vi "test_PinAndPinGroupContainingSamePin_ReserveSessions_ChannelMappingsDoesNotContainDuplicatePins.vi"() -> (6 "pass":bool, 8 "result":string, 15 "error out":errorcluster)   [LabVIEW 2021, in "MeasurementServerTests.lvlib" / "Session Reservation Tests.lvlib"]
uses:
  Session Reservation Tests.lvlib
  gRPC/Generated APIs/ni/measurementlink/sessionmanagement/v1/RPC Messages/ni_measurementlink_PinMapContext.ctl
  gRPC/Generated APIs/ni/measurementlink/sessionmanagement/v1/RPC Messages/ni_measurementlink_sessionmanagement_v1_ChannelMapping.ctl
  Runtime/Clients/Session Management V1/Session Reservation/Session Reservation.lvclass/Session Reservation.ctl
  3347d1b6-dca7-4e1a-9ca0-c9ec2f5aba95.vi
  ab61e54b-70f9-4719-86d2-c3025959eeb5.vi
  Runtime/Clients/Session Management V1/Session Reservation/Merge Invalid DVR Error.vi
  Runtime/Clients/Session Management V1/Session Reservation/Is DVR Valid.vi
  Runtime/Measurements/Helpers/Error Strings Global Internal.vi
  <vilib>/Utility/error.llb/Error Cluster From Error Code.vi
  <vilib>/JDP Science/JSONtext/Variant to JSON Text.vi
  <vilib>/JDP Science/JSONtext/LVClass Serializer/JSONtext LVClass Serializer.lvclass
  gRPC/Generated APIs/ni/measurementlink/sessionmanagement/v1/ni.measurementlink.sessionmanagement.v1.api.lvlib
  MeasurementServerTests.lvlib
  Runtime/Clients/Session Management V1/Session Reservation/Session Reservation.lvclass
panel:
  # "Test assumes discovery service, pin map service, and session management service have already been started."
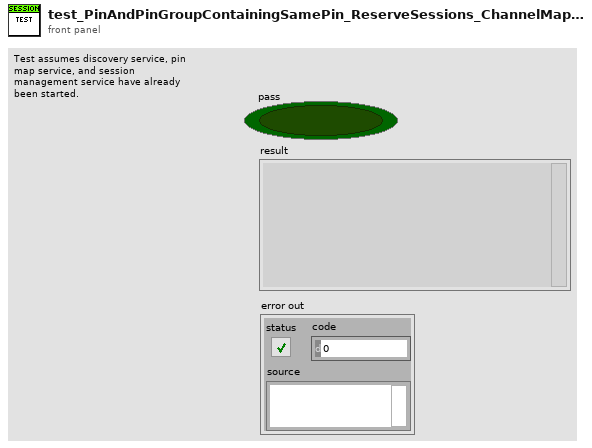
[diagram p1: front panel]
types:
  T1 = typedef "ni.measurementlink.sessionmanagement.v1.api.lvlib/ni_measurementlink_sessionmanagement_v1_ChannelMapping.ctl" = cluster{"pin_or_relay_name":string, "site":i32, "channel":string, "multiplexer_resource_name":string, "multiplexer_route":string}
  T2 = typedef "ni.measurementlink.sessionmanagement.v1.api.lvlib/ni_measurementlink_PinMapContext.ctl" = cluster{"pin_map_id":string, "sites":i32[]}
  T3 = typedef "ni.measurementlink.sessionmanagement.v1.api.lvlib/ni_measurementlink_sessionmanagement_v1_SessionInformation.ctl" = cluster{"session":T4, "resource_name":string, "channel_list":string, "instrument_type_id":string, "session_exists":bool, "session_reserved":bool, "channel_mappings":T1[], "annotations":T5[]}
  T4 = typedef "ni.measurementlink.sessionmanagement.v1.api.lvlib/nidevice_grpc_Session.ctl" = cluster{"name":string}
  T5 = typedef "ni.measurementlink.sessionmanagement.v1.api.lvlib/ni_measurementlink_sessionmanagement_v1_SessionInformation_AnnotationsEntry.ctl" = cluster{"key":string, "value":string}
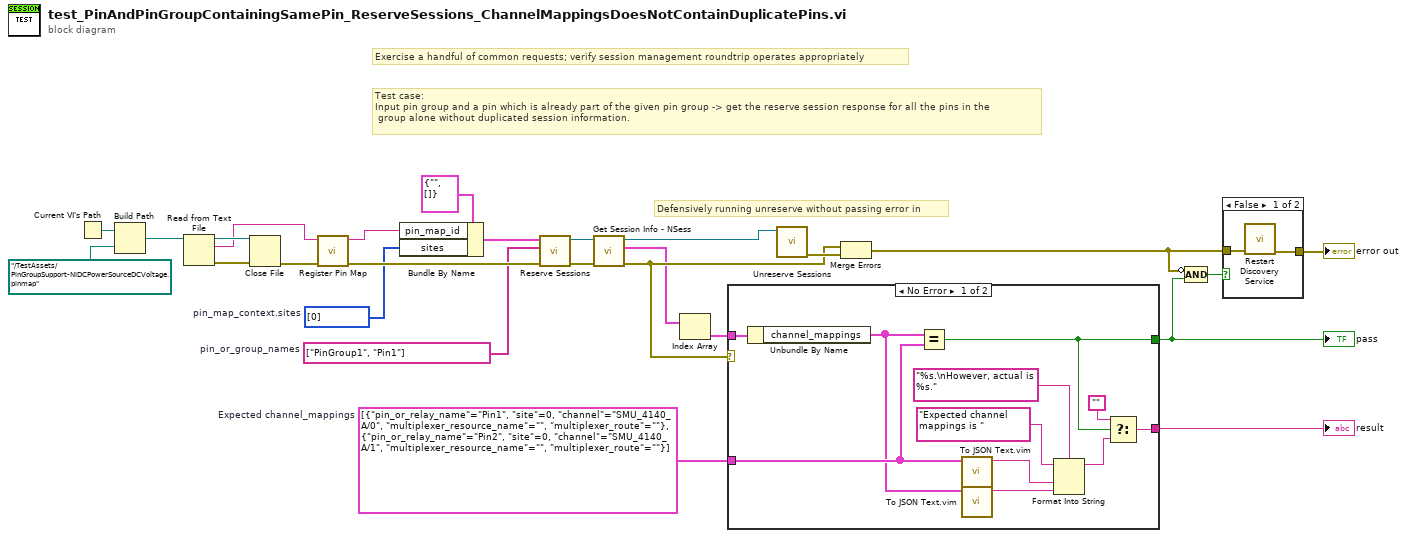
[diagram p0: block diagram]
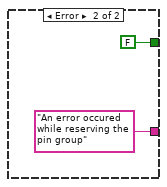
[diagram p3: hidden frame]
diagram:
  w5 = T1[] [{"pin_or_relay_name"="Pin1", "site"=0, "channel"="SMU_4140_A/0", "multiplexer_resource_name"="", "multiplexer_route"=""}, {"pin_or_relay_name"="Pin2", "site"=0, "channel"="SMU_4140_A/1", "multiplexer_resource_name"="", "multiplexer_route"=""}]  # Expected channel_mappings
  w10 = i32[] [0]  # pin_map_context.sites
  w9 = string[] ["PinGroup1", "Pin1"]  # pin_or_group_names
  # "Defensively running unreserve without passing error in"
  # "Test case:\nInput pin group and a pin which is already part of the given pin group -> get the reserve session response for all the pins in the\n\tgroup alone without duplicated session information."
  # "Exercise a handful of common requests; verify session management roundtrip operates appropriately"
  n1 = Current VI's Path() -> (path=w26:path)
  n2 = Build Path(base path=w26, name or relative path=path "../TestAssets/PinGroupSupport-NIDCPowerSourceDCVoltage.pinmap") -> (appended path=w24:path)
  n3 = Read from Text File(file (use dialog)=w24) -> (refnum out=w22:refnum<file>, text=w20:string, error out=w23:errorcluster)  [unwired: 3 in, 1 out]
  n4 = Close File(refnum=w22, error in=w23) -> (error out=w8:errorcluster)  [unwired: 1 out]
  n5 = call "Register Pin Map.vi"("error in"=w8, "pin map xml"=w20) -> ("error out"=w12:errorcluster, "pin map id"=w11:string)  [unwired: 8 in]
  n6 = Bundle By Name(cluster=T2 {"pin_map_id"="", "sites"=[]} ("pin map context"), "pin_map_id"=w11, "sites"=w10) -> (w19:T2)
  n7 = call "Reserve Sessions.vi"("error in"=w12, "pin or relay names"=w9, "pin map context"=w19) -> ("error out"=w18:errorcluster, "session reservation out"=w17:refnum<class "Session Reservation.lvclass">)  [unwired: 7 in]
  n8 = call "Get Session Info - NSess .vi"("error in"=w18, "session reservation in"=w17) -> ("error out"=w13:errorcluster, "sessions info"=w7:T3[], "session reservation out"=w6:refnum<class "Session Reservation.lvclass">)  [unwired: 7 in]
  n9 = Index Array(array=w7) -> (element=w1:T3)  [unwired: 1 in]
  n10 = case shown="No Error" w13 {
    tunnel: [w32 FALSE] -> w4
    tunnel: w5 -> [w33 _]
    tunnel: [w30 "An error occured while reserving the pin group" ("String")] -> w2
    tunnel: w1 -> [w27 _]
    frame No Error {
      n11 = Unbundle By Name(w27) -> ("channel_mappings"=w28:T1[])
      n12 = Equal?(x=w28, y=w33) -> (x = y?=w32:bool)
      n13 = call "To JSON Text.vim"("Anything"=w33) -> ("<JSON>"=w36:string)  [unwired: 9 in, 1 out]
      n14 = call "To JSON Text.vim"("Anything"=w28) -> ("<JSON>"=w35:string)  [unwired: 9 in, 1 out]
      n15 = Format Into String(format string="%s.\nHowever, actual is %s.", initial string="Expected channel mappings is ", w36, w35) -> (resulting string=w34:string)  [unwired: 1 in, 1 out]
      n16 = Select(t="", s=w32, f=w34) -> (s? t:f=w30:string)
    }
    frame Error {
    }
  }
  "pass" <- w4
  "result" <- w2
  n17 = call "Unreserve Sessions.vi"("session reservation in"=w6) -> ("error out"=w16:errorcluster)  [unwired: 10 in]
  n18 = Merge Errors(w13, w16) -> (w14:errorcluster)
  n19 = Compound Arithmetic op=AND(invert w14, w4) -> (w15:bool)
  n20 = case shown="False" w15 {
    tunnel: [w41 w42] -> w3
    tunnel: w14 -> [w40 w42]
    frame False {
      n21 = call "Restart Discovery Service.vi"("error in"=w40) -> ("error out"=w41:errorcluster)  [unwired: 10 in]
    }
    frame True {
    }
  }
  "error out" <- w3
